vi "Configure - Analog.vi"(7 "DAQmx Physical Channel":tag="PXI1Slot4/ao0", 8 "error in (no error)":errorcluster, 9 "signal settings":T3, 10 "output settings":T1={"output rate"=0.0, "range"=0.0, "terminal configuration"=enum."Pseudodifferential", "output impedance"=0.0, "common mode offset"=0.0, "pure tone mode"=FALSE}, 11 "AudioGeneration in":refnum<class "AudioGeneration.lvclass">) -> (0 "error out":errorcluster, 3 "AudioGeneration out":refnum<class "AudioGeneration.lvclass">)   [LabVIEW 2021, in "AudioGeneration.lvclass"]
uses:
  AudioGeneration.lvclass
  AudioGeneration.lvclass/AudioGeneration.ctl
  <vilib>/NI/STM/TCP/TCP Write Options.ctl
  <vilib>/NI/STM/NI STM.lvlib
  controls/generation type.ctl
  controls/AudioGenTypeDefs.lvlib
  <vilib>/NI/STM/TCP/Write Message (TCP).vi
  controls/terminal configuration.ctl
  controls/analog output settings.ctl
  controls/signal type.ctl
  controls/signal settings.ctl
  controls/analog generation settings.ctl
panel:
  out "timeout":bool
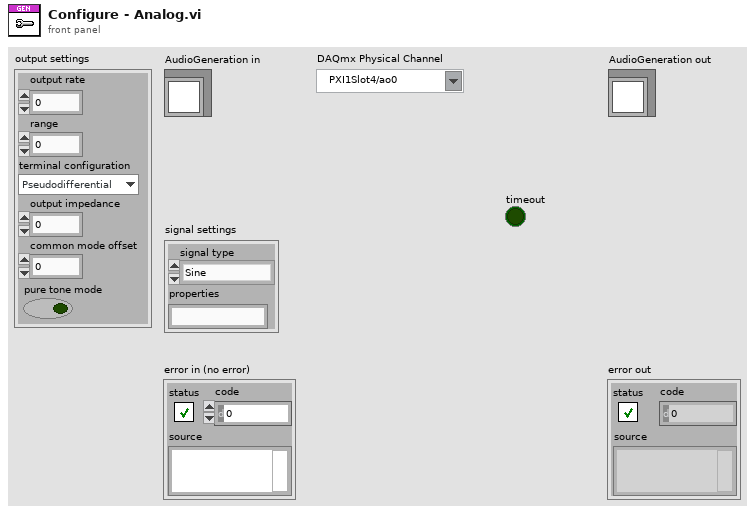
[diagram p1: front panel]
types:
  T1 = typedef "AudioGenTypeDefs.lvlib/analog output settings.ctl" = cluster{"output rate":dbl, "range":dbl, "terminal configuration":T2, "output impedance":dbl, "common mode offset":dbl, "pure tone mode":bool}
  T2 = typedef "AudioGenTypeDefs.lvlib/terminal configuration.ctl" = enum32{"Default", "RSE", "Differential", "Pseudodifferential"}
  T3 = typedef "AudioGenTypeDefs.lvlib/signal settings.ctl" = cluster{"signal type":T4, "properties":string}
  T4 = typedef "AudioGenTypeDefs.lvlib/signal type.ctl" = enum16{"Sine", "Square", "Triangle", "White Noise", "Pink Noise", "Periodic Random Noise"}
  T5 = typedef "AudioGenTypeDefs.lvlib/analog generation settings.ctl" = cluster{"channel list":string, "output settings":T1, "signal settings":T3}
  T6 = typedef "AudioGenTypeDefs.lvlib/generation type.ctl" = enum16{"analog", "digital"}
  T7 = typedef "NI STM.lvlib/TCP Write Options.ctl" = cluster{"ignore timeout error":bool, "timeout ms (1000)":i32}
  T8 = typedef "NI STM.lvlib/TCP Connection Info.ctl" = cluster{"connection ID":refnum<k5>, "meta data":T9[]}
  T9 = typedef "NI STM.lvlib/MetaDataElement.ctl" = string
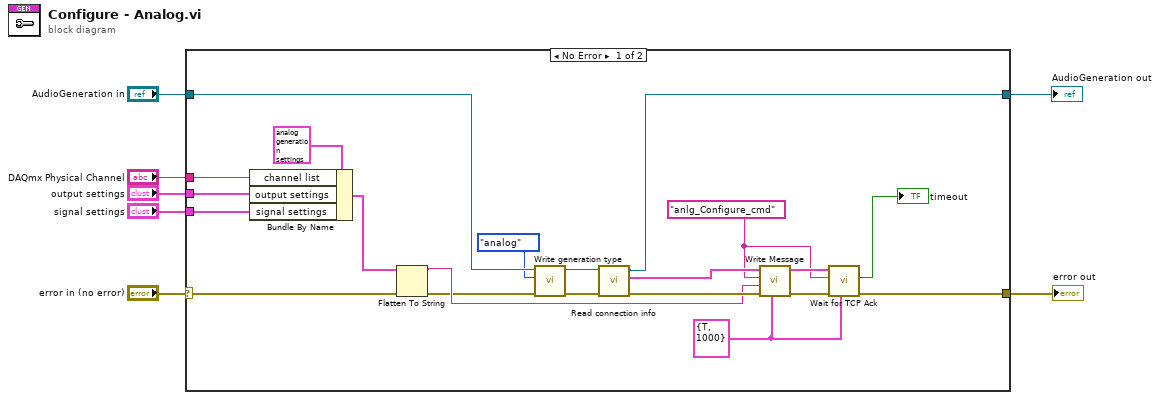
[diagram p0: block diagram]
diagram:
  n1 = case shown="No Error" "error in (no error)" {
    selector: "error in (no error)" -> [w23 w30]
    tunnel: [w25 w30] -> w5
    tunnel: "AudioGeneration in" -> [w18 w29]
    tunnel: [w24 w29] -> w4
    tunnel: "output settings" -> [w11 _]
    tunnel: "signal settings" -> [w10 _]
    tunnel: "DAQmx Physical Channel" -> [w9 _]
    frame No Error {
      w14 = "anlg_Configure_cmd" ("name")
      w15 = T7 {"ignore timeout error"=TRUE, "timeout ms (1000)"=1000} ("options")
      n2 = Bundle By Name(cluster=T5 {"channel list"="", "output settings"={"output rate"=0.0, "range"=0.0, "terminal configuration"=enum."Pseudodifferential", "output impedance"=0.0, "common mode offset"=0.0, "pure tone mode"=FALSE}, "signal settings"={"signal type"=enum."Sine", "properties"=""}} ("analog generation"), "channel list"=w9, "output settings"=w11, "signal settings"=w10) -> (w12:T5)
      n3 = Flatten To String(anything=w12, error in (no error)=w23) -> (data string=w22:string, error out=w21:errorcluster)  [unwired: 2 in, 1 out]
      n4 = call-dynamic "Write generation type.vi"("error in (no error)"=w21, "generation type"=generation_type."analog", "AudioGeneration in"=w18) -> ("error out"=w20:errorcluster, "AudioGeneration out"=w19:refnum<class "AudioGeneration.lvclass">)  [unwired: 7 in]
      n5 = call-dynamic "Read connection info.vi"("error in (no error)"=w20, "AudioGeneration in"=w19) -> ("error out"=w27:errorcluster, "connection info"=w28:T8, "AudioGeneration out"=w24:refnum<class "AudioGeneration.lvclass">)  [unwired: 7 in]
      n6 = call-poly <vilib>:"Write Message.vi"("options"=w15, "error in"=w27, "data"=w22, "name"=w14, "connection info in"=w28) -> ("error out"=w26:errorcluster, "connection info out"=w16:T8)  [unwired: 5 in]
      n7 = call "Wait for TCP Ack.vi"("options"=w15, "error in (no error)"=w26, "cmd name"=w14, "connection info in"=w16) -> ("error out"=w25:errorcluster, "timeout"=→"timeout":bool)  [unwired: 4 in, 2 out]
    }
    frame Error {
    }
  }
  "error out" <- w5
  "AudioGeneration out" <- w4
